vi "get Permit Range Frequency.vi"(8 "error in (no error)":errorcluster, 10 "Trace Values":T1 {"Frequency" format="%#_6p"}, 11 "SA Measurement in":refnum<class "SA Measurement.lvclass">) -> (0 "error out":errorcluster, 3 "SA Measurement out":refnum<class "SA Measurement.lvclass">)   [LabVIEW 2023, in "Spectrum Analyzer.lvlib" / "SA Measurement.lvclass"]
uses:
  SA Measurement.lvclass
  SA Measurement.lvclass/SA Measurement.ctl
  TYPE DEFINITION/TYPE Trace Value Array.ctl
  Spectrum Analyzer.lvlib
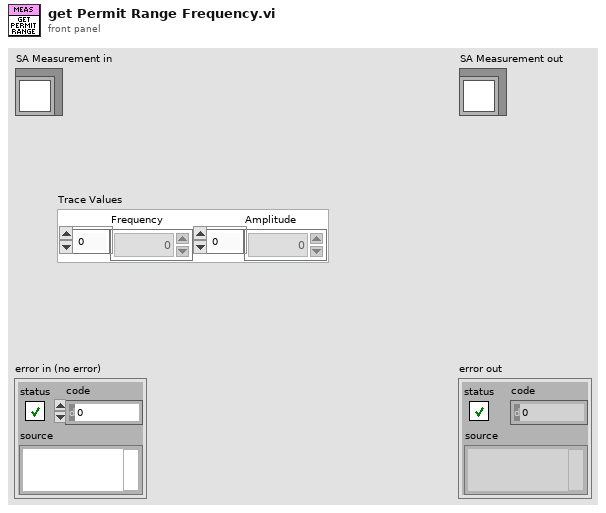
[diagram p1: front panel]
types:
  T1 = typedef "Spectrum Analyzer.lvlib/TYPE Trace Value Array.ctl" = cluster{"Frequency":dbl[], "Amplitude":dbl[]}
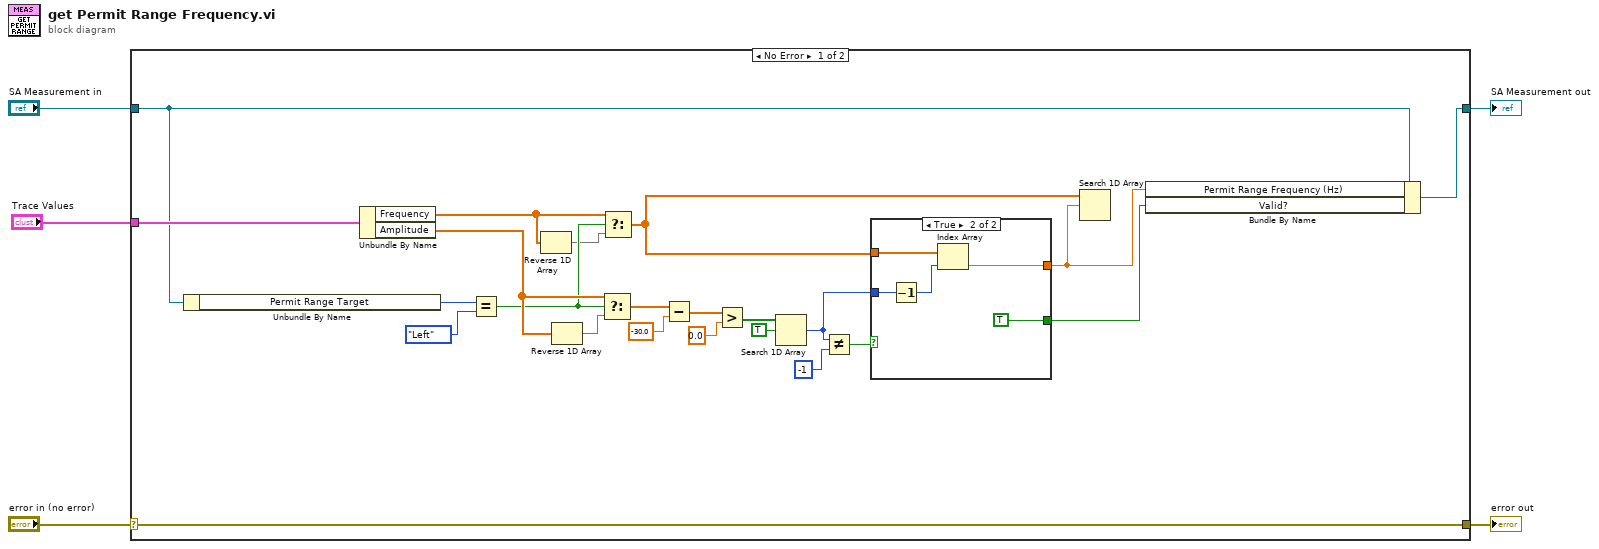
[diagram p0: block diagram]
diagram:
  n1 = case shown="No Error" "error in (no error)" {
    selector: "error in (no error)" -> [w28 w35]
    tunnel: [w28 w35] -> w4
    tunnel: [w8 w34] -> w2
    tunnel: "SA Measurement in" -> [w10 w34]
    tunnel: "Trace Values" -> [w27 _]
    frame No Error {
      n2 = Unbundle By Name(w10) -> ("Permit Range Target"=w20:enum16{"Left", "Right"})
      n3 = Unbundle By Name(w27) -> ("Frequency"=w15:dbl[], "Amplitude"=w17:dbl[])
      n4 = Equal?(x=w20, y=enum16{"Left", "Right"}."Left") -> (x = y?=w16:bool)
      n5 = Reverse 1D Array(array=w15) -> (reversed array=w14:dbl[])
      n6 = Reverse 1D Array(array=w17) -> (reversed array=w18:dbl[])
      n7 = Select(t=w17, s=w16, f=w18) -> (s? t:f=w13:dbl[])
      n8 = Select(t=w15, s=w16, f=w14) -> (s? t:f=w9:dbl[])
      n9 = Subtract(x=w13, y=-30.0) -> (x-y=w25:dbl[])
      n10 = Greater?(x=w25, y=0.0) -> (0:w23:bool[])
      n11 = Search 1D Array(1D array=w23, element=TRUE) -> (index of element=w11:i32)  [unwired: 1 in]
      n12 = Not Equal?(x=w11, y=-1) -> (x != y?=w12:bool)
      n13 = case shown="True" w12 {
        tunnel: w9 -> [_ w33]
        tunnel: w11 -> [_ w32]
        tunnel: [_ w30] -> w7
        tunnel: [_ TRUE] -> w6
        frame False {
        }
        frame True {
          n14 = Decrement(x=w32) -> (x-1=w31:i32)
          n15 = Index Array(array=w33, index=w31) -> (element=w30:dbl)
        }
      }
      n16 = Search 1D Array(1D array=w9, element=w7) -> ()  [unwired: 1 in, 1 out]
      n17 = Bundle By Name(cluster=w10, "Permit Range Frequency (Hz)"=w7, "Valid?"=w6) -> (w8:refnum<class "SA Measurement.lvclass">)
    }
    frame Error {
    }
  }
  "error out" <- w4
  "SA Measurement out" <- w2
